vi "Create.vi"(8 "error in":errorcluster, 10 "Parent Reference":refnum<vi>, 11 "Element Array in":refnum<class "Array.lvclass">) -> (0 "error out":errorcluster, 3 "Element Array out":refnum<class "Array.lvclass">)   [LabVIEW 2026, in "Array.lvclass"]
doc: "Create Element."
uses:
  Array.lvclass
  <vilib>/Utility/miscctls.llb/LVPointTypeDef.ctl
  Array.lvclass/Array.ctl
  Interfaces/IElement/IElement.lvclass
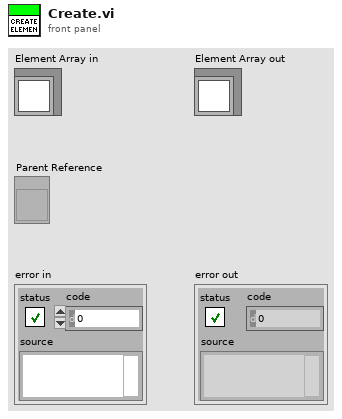
[diagram p1: front panel]
types:
  T1 = typedef "LVPointTypeDef.ctl" = cluster{"Horizontal":i16, "Vertical":i16}
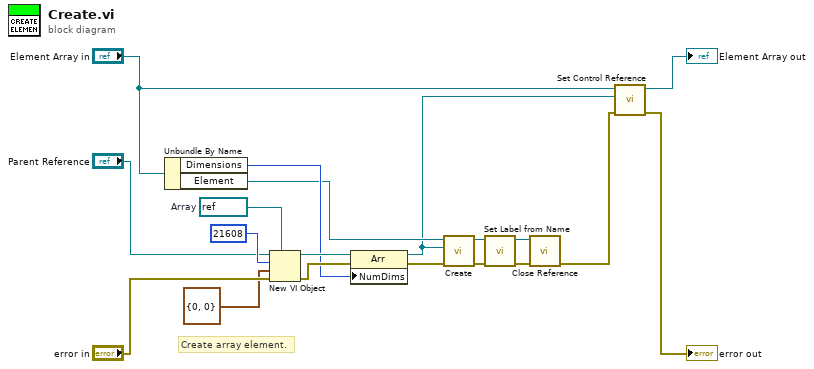
[diagram p0: block diagram]
diagram:
  w15 = refnum<vi> refnum  # Array
  # "Create array element."
  n1 = Unbundle By Name("Element Array in") -> ("Dimensions"=w11:i32, "Element"=w9:refnum<class "IElement.lvclass">)
  n2 = New VI Object(vi object class=w15, owner refnum="Parent Reference", style=u32 21608, position/next to=T1 {"Horizontal"=0, "Vertical"=0} ("location"), 8:"error in") -> (object refnum=w14:refnum<vi>, 0:w19:errorcluster)  [unwired: 3 in]
  n3 = property on="Property Node" class="Arr"(reference=w14, error in=w19, "NumDims"=w11) -> (reference out=w6:refnum<vi>, error out=w17:errorcluster)
  n4 = call-dynamic "Create.vi"("error in"=w17, "Parent Reference"=w6, "IElement in"=w9) -> ("error out"=w2:errorcluster, "IElement out"=w5:refnum<class "IElement.lvclass">)  [unwired: 7 in]
  n5 = call-dynamic "Set Label from Name.vi"("error in"=w2, "IElement in"=w5) -> ("error out"=w3:errorcluster, "IElement out"=w4:refnum<class "IElement.lvclass">)  [unwired: 8 in]
  n6 = call-dynamic "Close Reference.vi"("error in"=w3, "IElement in"=w4) -> ("error out"=w1:errorcluster)  [unwired: 8 in, 1 out]
  n7 = call-dynamic "Set Control Reference.vi"("error in"=w1, "Control Reference"=w6, "Element in"="Element Array in") -> ("error out"=→"error out":errorcluster, "Element out"=→"Element Array out":refnum<class "Array.lvclass">)  [unwired: 7 in]
